vi "PeriodicFilter-Update Filtered Info.vi"(7 "Seconds Since 1Jan1904":timestamp, 8 "Settings":T1={"threashold(#/s)"=1.0, "Check Peroid(s)"=1.0}, 11 "Data In":T2 {"LastCheckT" format="%<%.3X>T"}) -> (3 "Data Out":T2 {"LastCheckT" format="%<%.3X>T"})   [LabVIEW 2017, in "Communicable State Machine.lvlib"]
uses:
  Communicable State Machine.lvlib
  Periodic String Filter Data.ctl
  Periodic String Filter Info.ctl
  Periodic String Filter Setting.ctl
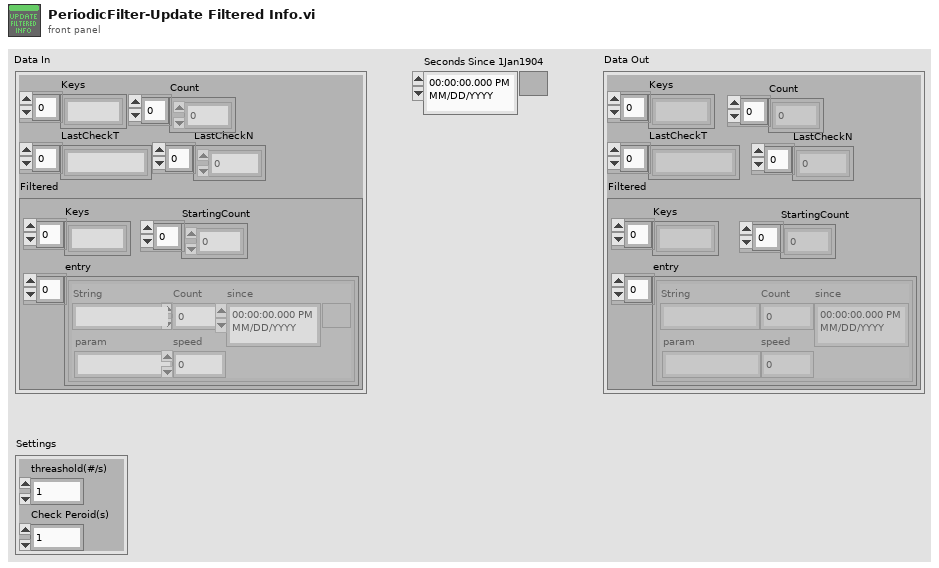
[diagram p1: front panel]
types:
  T1 = typedef "Communicable State Machine.lvlib/Periodic String Filter Setting.ctl" = cluster{"threashold(#/s)":dbl, "Check Peroid(s)":dbl}
  T2 = typedef "Communicable State Machine.lvlib/Periodic String Filter Data.ctl" = cluster{"Keys":string[], "Count":i64[], "LastCheckT":timestamp[], "LastCheckN":i64[], "Filtered":cluster{"Keys":string[], "StartingCount":i64[], "entry":T3[]}}
  T3 = typedef "Communicable State Machine.lvlib/Periodic String Filter Info.ctl" = cluster{"String":string, "Count":i64, "since":timestamp, "param":string, "speed":dbl}
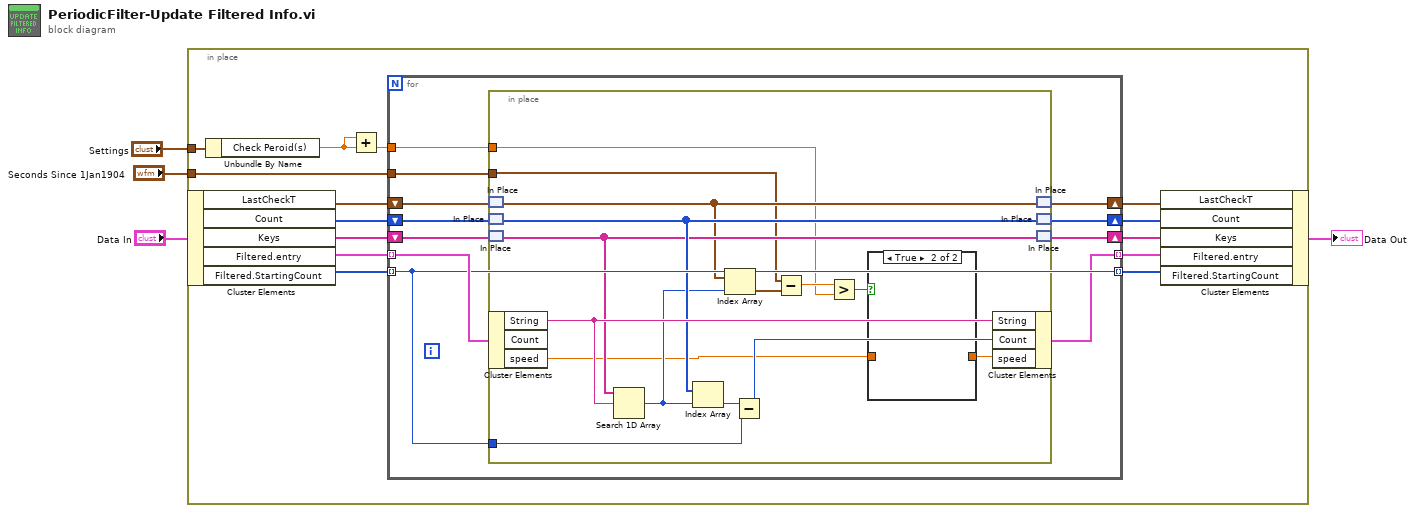
[diagram p0: block diagram]
diagram:
  n1 = in-place "In Place Element Structure" {
    in-place-border: "Seconds Since 1Jan1904" -> [w10]
    in-place-border: "Settings" -> [w7]
    n2 = in-place-cluster #1("Data In") -> ("LastCheckT"=w9:timestamp[], "Count"=w16:i64[], "Keys"=w18:string[], "Filtered.entry"=w14:T3[], "Filtered.StartingCount"=w13:i64[])
    n3 = Unbundle By Name(w7) -> ("Check Peroid(s)"=w5:dbl)
    n4 = Add(x=w5, y=w5) -> (x+y=w6:dbl)
    n5 = for {
      shift-right: [w21] -> w17
      shift-left: w18 -> [w22]
      shift-right: [w23] -> w15
      shift-left: w16 -> [w24]
      tunnel: w14 -> [w29] mode=indexing
      tunnel: w13 -> [w28] mode=indexing
      tunnel: [w28] -> w12 mode=indexing
      tunnel: [w27] -> w11 mode=indexing
      tunnel: w10 -> [w20]
      shift-right: [w25] -> w8
      shift-left: w9 -> [w26]
      tunnel: w6 -> [w19]
      n6 = in-place {
        in-place-border: w28 -> [w43]
        in-place-border: w20 -> [w34]
        in-place-border: w19 -> [w33]
        n7 = in-place-match #2(w26) -> (w38:timestamp[])
        n8 = in-place-match #3(w24) -> (w40:i64[])
        n9 = in-place-match #4(w22) -> (w39:string[])
        n10 = in-place-cluster #5(w29) -> ("String"=w41:string, "speed"=w30:dbl)  [unwired: 1 out]
        n11 = Search 1D Array(1D array=w39, element=w41) -> (index of element=w37:i32)  [unwired: 1 in]
        n12 = Index Array(array=w40, index=w37) -> (element=w44:i64)
        n13 = Index Array(array=w38, index=w37) -> (element=w35:timestamp)
        n14 = Subtract(x=w44, y=w43) -> (x-y=w42:i64)
        n15 = Subtract(x=w34, y=w35) -> (x-y=w36:dbl)
        n16 = Greater?(x=w36, y=w33) -> (0:w32:bool)
        n17 = case shown="True" w32 {
          tunnel: [w45 _] -> w31
          tunnel: w30 -> [w45 _]
          frame False {
          }
          frame True {
          }
        }
        n18 = in-place-cluster #5("String"=w41, "Count"=w42, "speed"=w31) -> (w27:T3)
        n19 = in-place-match #2(w38) -> (w25:timestamp[])
        n20 = in-place-match #3(w40) -> (w23:i64[])
        n21 = in-place-match #4(w39) -> (w21:string[])
      }
    }
    n22 = in-place-cluster #1("LastCheckT"=w8, "Count"=w15, "Keys"=w17, "Filtered.entry"=w11, "Filtered.StartingCount"=w12) -> (→"Data Out":T2)
  }
